vi "getXMLHeader.vi"(11 "Test Report in":refnum<class "Test Report.JUnit.lvclass">) -> (2 "xml header":string)   [LabVIEW 2020, in "Caraya.lvlib" / "Test Report.JUnit.lvclass"]
uses:
  Test Report.JUnit.lvclass
  C:/projects/caraya/src/classes/Test Report/Test Report.lvclass
  Test Report/Test Report.lvclass/Test Report.ctl
  MsgSerializer/MsgSerializer.lvclass/MsgSerializer.ctl
  MsgSerializer/MsgSerializer.lvclass
  MsgSerializer.XML/MsgSerializer.XML.lvclass
  Test Report/Test Report.lvclass
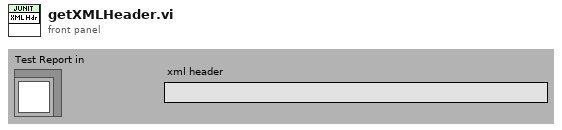
[diagram p1: front panel]
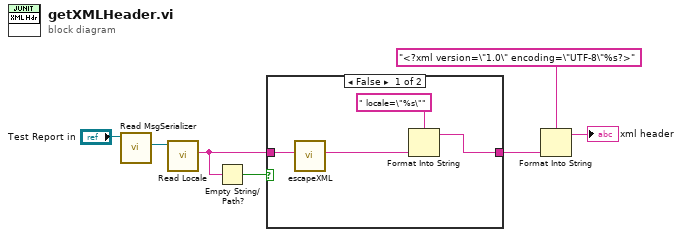
[diagram p0: block diagram]
diagram:
  n1 = call "Read MsgSerializer.vi"("Test Report in"="Test Report in") -> ("MsgSerializer"=w1:refnum<class "MsgSerializer.lvclass">)  [unwired: 9 in, 1 out]
  n2 = call "Read Locale.vi"("MsgSerializer"=w1) -> ("Locale"=w7:string)  [unwired: 9 in, 1 out]
  n3 = Empty String/Path?(string/path=w7) -> (empty?=w6:bool)
  n4 = case shown="False" w6 {
    tunnel: w7 -> [w11 _]
    tunnel: [w9 _] -> w5
    frame False {
      n5 = call "escapeXML.vi"("Input String"=w11) -> ("XML-escaped String"=w10:string)  [unwired: 10 in]
      n6 = Format Into String(format string=" locale=\"%s\"", w10) -> (resulting string=w9:string)  [unwired: 2 in, 1 out]
    }
    frame True {
    }
  }
  n7 = Format Into String(format string="<?xml version=\"1.0\" encoding=\"UTF-8\"%s?>" ("xml header"), w5) -> (resulting string=→"xml header":string)  [unwired: 2 in, 1 out]
